vi "PicoScope6000aIsReady.vi"(8 "error in (no error)":errorcluster, 11 "handle in":i16) -> (0 "error out":errorcluster, 3 "handle out":i16, 6 "ready":i16)   [LabVIEW 2009]
doc: "Calls ps6000aIsReady"
uses:
  ps6000a.dll
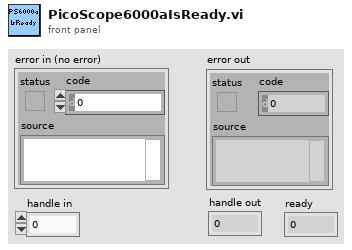
[diagram p1: front panel]
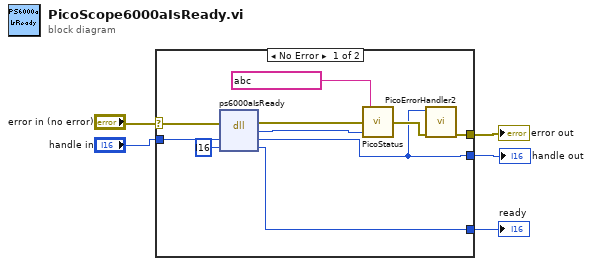
[diagram p0: block diagram]
diagram:
  n1 = case shown="No Error" "error in (no error)" {
    selector: "error in (no error)" -> [w14 w16]
    tunnel: "handle in" -> [w15 w17]
    tunnel: [w8 w17] -> w5
    tunnel: [w9 w16] -> w4
    tunnel: [w6 _] -> w3
    frame #0 {
      n2 = dll-call lib="ps6000a.dll" fn="ps6000aIsReady" ("ps3000.dll:_ps3000_open_unit@0")(error in=w14, "handle"=w15, "ready"=i16 ?) -> (error out=w13:errorcluster, "PICO_STATUS"=w12:u32, "handle"=w8:i16, "ready"=w6:i16)  [unwired: 2 in, 1 out]
      n3 = call "PicoStatus.vi"("PICO STATUS"=w12, "error in"=w13, "source"=string ?) -> ("error out"=w10:errorcluster)
      n4 = call "PicoErrorHandler2.vi"("error in (no error)"=w10, "handle In"=w8) -> ("error out"=w9:errorcluster)  [unwired: 9 in]
    }
    frame #1 {
    }
  }
  "error out" <- w4
  "handle out" <- w5
  "ready" <- w3
